vi "Should Update Channel.vi"(7 "Connected?":bool, 10 "Address":i32, 11 "Valid?":bool) -> (3 "Update?":bool)   [LabVIEW 2026, in "Modbus.lvlib" / "Modbus.lvclass"]
uses:
  Modbus.lvclass
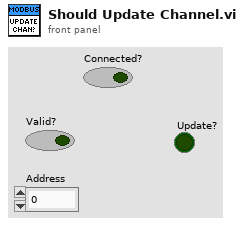
[diagram p1: front panel]
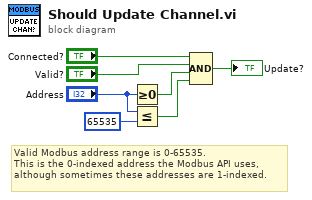
[diagram p0: block diagram]
diagram:
  # "Valid Modbus address range is 0-65535.\nThis is the 0-indexed address the Modbus API uses,\nalthough sometimes these addresses are 1-indexed."
  n1 = Greater Or Equal To 0?(x="Address") -> (x >= 0?=w5:bool)
  n2 = Less Or Equal?(x="Address", y=65535 ("Address")) -> (x <= y?=w2:bool)
  n3 = Compound Arithmetic op=AND("Connected?", "Valid?", w5, w2) -> (→"Update?":bool)
